vi "Close.vi"(8 "error in (no error)":errorcluster, 9 "Stop Event":refnum<user-event>, 10 "Sequence Context":refnum<k7>, 11 "Abstract":refnum<class "Abstract.lvclass">=refnum) -> (0 "error out":errorcluster, 3 "Abstract out":refnum<class "Abstract.lvclass">)   [LabVIEW 2025, in "Abstract.lvclass"]
uses:
  Abstract.lvclass
  Abstract.lvclass/Abstract.ctl
  <vilib>/OPCUA/NI OPC UA Client.lvlib
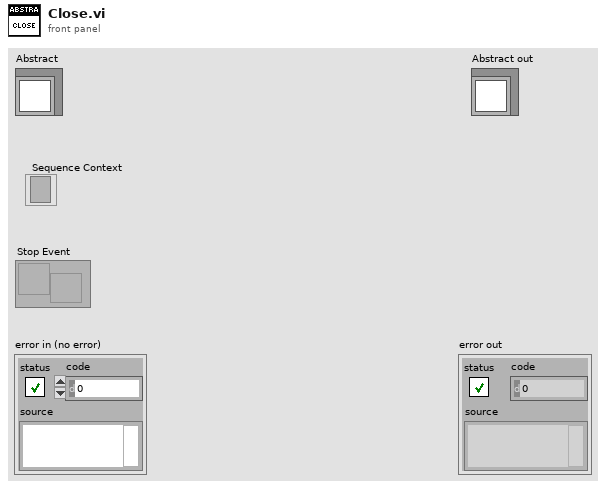
[diagram p1: front panel]
types:
  T1 = typedef "OPC UA Client Refnum.ctl" = refnum<k21>
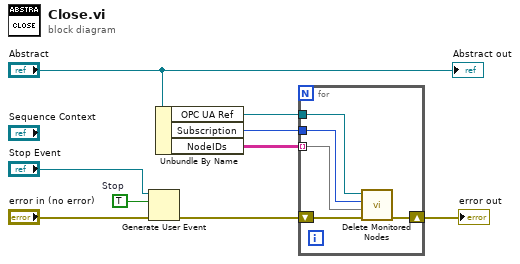
[diagram p0: block diagram]
diagram:
  w4 = TRUE  # Stop
  n1 = Generate User Event(user event="Stop Event", event data cluster=w4, error in="error in (no error)") -> (error out=w2:errorcluster)  [unwired: 1 in, 1 out]
  n2 = Unbundle By Name("Abstract") -> ("OPC UA Ref"=w8:T1, "Subscription"=w7:u32, "NodeIDs"=w6:string[][])
  n3 = for {
    shift-right: [w14] -> w9
    shift-left: w2 -> [w13]
    tunnel: w8 -> [w12]
    tunnel: w6 -> [w11] mode=indexing
    tunnel: w7 -> [w10]
    n4 = call <vilib>:"Delete Monitored Nodes.vi"("error in (no error)"=w13, "node IDs"=w11, "subscription ID in"=w10, "OPC UA client refnum in"=w12) -> ("error out"=w14:errorcluster)  [unwired: 3 in, 4 out]
  }
  "error out" <- w9
  "Abstract out" <- "Abstract"
